vi "Set Control Reference.vi"(8 "error in":errorcluster, 10 "Control Reference":refnum<vi>, 11 "Element in":refnum<class "Element.lvclass">) -> (0 "error out":errorcluster, 3 "Element out":refnum<class "Element.lvclass">)   [LabVIEW 2026, in "Element.lvclass"]
doc: "Set Control Reference."
uses:
  Element.lvclass
  Element.lvclass/Element.ctl
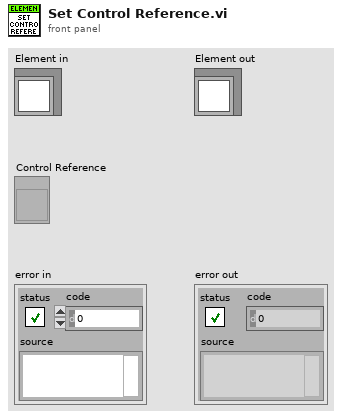
[diagram p1: front panel]
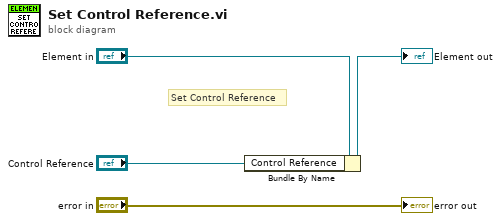
[diagram p0: block diagram]
diagram:
  # "Set Control Reference"
  n1 = Bundle By Name(cluster="Element in", "Control Reference"="Control Reference") -> (→"Element out":refnum<class "Element.lvclass">)
  "error out" <- "error in"
